vi "Disable Frame10 Enabled.vi"(8 "error in":errorcluster) -> (0 "error out":errorcluster, 1 "Result":i32)   [LabVIEW 2026]
doc: "Issue 129 repro: twelve frames, frame 10 enabled, so activeDiag reads 0A."
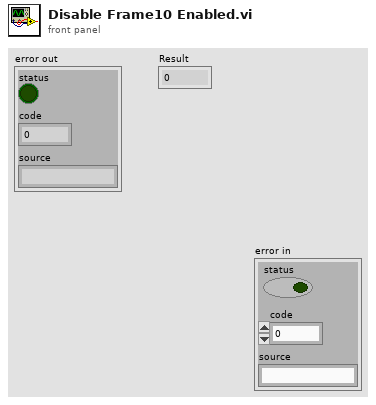
[diagram p1: front panel]
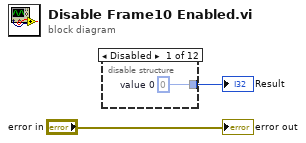
[diagram p0: block diagram]
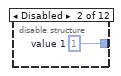
[diagram p2: hidden frame]
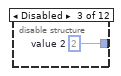
[diagram p3: hidden frame]
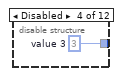
[diagram p4: hidden frame]
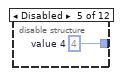
[diagram p5: hidden frame]
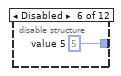
[diagram p6: hidden frame]
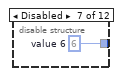
[diagram p7: hidden frame]
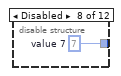
[diagram p8: hidden frame]
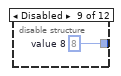
[diagram p9: hidden frame]
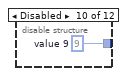
[diagram p10: hidden frame]
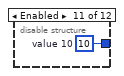
[diagram p11: hidden frame]
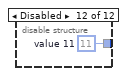
[diagram p12: hidden frame]
diagram:
  n1 = disable-structure shown="Disabled" {
    disable-tunnel: [w3 w4 w5 w6 w7 w8 w9 w10 w11 w12 w13 w14] -> w2
    frame Disabled {
      w3 = 0  # value 0
    }
    frame Disabled {
      w4 = 1  # value 1
    }
    frame Disabled {
      w5 = 2  # value 2
    }
    frame Disabled {
      w6 = 3  # value 3
    }
    frame Disabled {
      w7 = 4  # value 4
    }
    frame Disabled {
      w8 = 5  # value 5
    }
    frame Disabled {
      w9 = 6  # value 6
    }
    frame Disabled {
      w10 = 7  # value 7
    }
    frame Disabled {
      w11 = 8  # value 8
    }
    frame Disabled {
      w12 = 9  # value 9
    }
    frame Enabled {
      w13 = 10  # value 10
    }
    frame Disabled {
      w14 = 11  # value 11
    }
  }
  "Result" <- w2
  "error out" <- "error in"
